vi "UpdateLastTime.vi"(8 "error in (no error)":errorcluster, 11 "feed GUID":string) -> (0 "error out":errorcluster)   [LabVIEW 2023, in "GettingStartedWindow.lvlib" / "Feed_link.lvclass"]
uses:
  <resource>/modes/FRC/Classes/Feed_link/Feed_link.lvclass
  <vilib>/Utility/config.llb/NI_LVConfig.lvlib
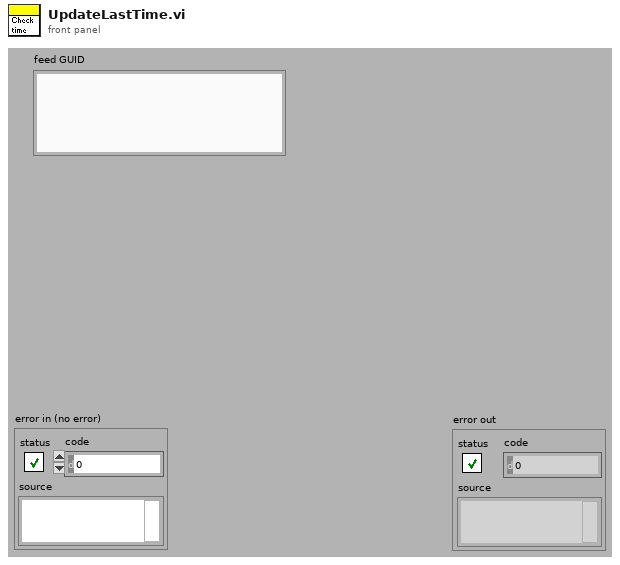
[diagram p1: front panel]
types:
  T1 = typedef "NI_LVConfig.lvlib/Config Data RefNum.ctl" = refnum<k1>
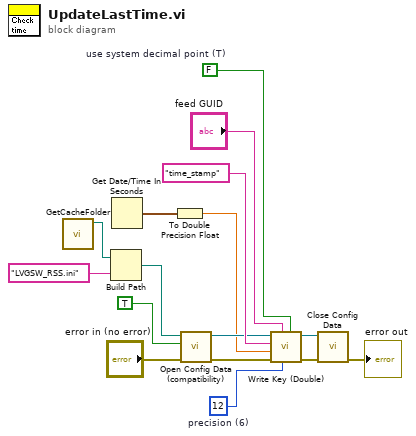
[diagram p0: block diagram]
diagram:
  w4 = i16 12  # precision (6)
  w5 = FALSE  # use system decimal point (T)
  n1 = call <resource>:"GetCacheFolder.vi"() -> ("cache folder"=w16:path)  [unwired: 1 in, 10 out]
  n2 = Build Path(base path=w16, name or relative path="LVGSW_RSS.ini") -> (appended path=w14:path)
  n3 = Get Date/Time In Seconds() -> (seconds since 1Jan1904=w11:timestamp)
  n4 = To Double Precision Float(number=w11) -> (double precision float=w1:dbl)
  n5 = call <vilib>:"Open Config Data (compatibility).vi"("error in (no error)"="error in (no error)", "create file if necessary (T)"=TRUE ("create file if necessary? (T)"), "configuration file path"=w14) -> ("error out"=w2:errorcluster, "refnum"=w3:T1)  [unwired: 6 in, 1 out]
  n6 = call <vilib>:"Write Key (Double).vi"("use system decimal point (T)"=w5, "precision (6)"=w4, "section"="feed GUID", "error in (no error)"=w2, "value"=w1, "key"="time_stamp", "refnum"=w3) -> ("error out"=w9:errorcluster, "refnum out"=w10:T1)  [unwired: 1 in, 2 out]
  n7 = call <vilib>:"Close Config Data.vi"("error in (no error)"=w9, "refnum"=w10) -> ("error out"=→"error out":errorcluster)  [unwired: 1 in, 8 out]
